vi "readText.vi"(8 "error in (no error)":errorcluster, 11 "MS-Word in":refnum<class "MS-Word.lvclass">) -> (0 "error out":errorcluster, 2 "Text":string, 3 "MS-Word out":refnum<class "MS-Word.lvclass">)   [LabVIEW 2017, in "LabVIEW NPOI.lvlib" / "MS-Word.lvclass"]
uses:
  MS-Word.lvclass
  MS-Word.lvclass/MS-Word.ctl
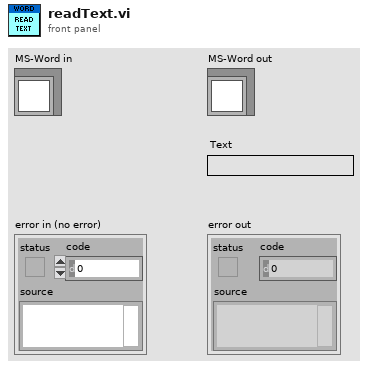
[diagram p1: front panel]
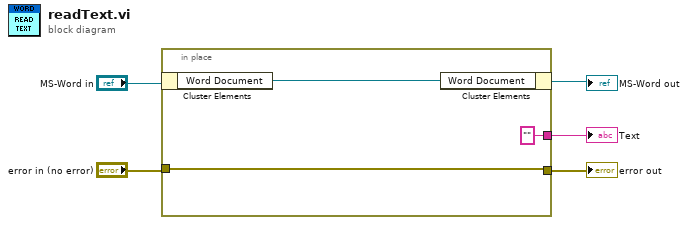
[diagram p0: block diagram]
diagram:
  n1 = in-place {
    in-place-border: "error in (no error)" -> [w8]
    in-place-border: [w8] -> w2
    in-place-border: ["" ("All Characters")] -> w1
    n2 = in-place-cluster #1("MS-Word in") -> ("Word Document"=w7:refnum<class "xwpfDocument.lvclass">)
    n3 = in-place-cluster #1("Word Document"=w7) -> (→"MS-Word out":refnum<class "MS-Word.lvclass">)
  }
  "error out" <- w2
  "Text" <- w1
